vi "Test Running Entry.vi"(8 "error in (no error)":errorcluster, 10 "Work Folder":path, 11 "Test Data Folder":path) -> (0 "error out":errorcluster, 2 "Report":string, 3 "Passed":bool)   [LabVIEW 2024]
doc: "A running entry has End Time 0 in memory and End Time = \"\" in the file. Saves an entry that started an hour ago with no end and checks that Get Running Entry returns it, that the file holds End Time = \"\" and that Read Entry gives End Time 0 back. Then checks the other direction with the README sample: its entry with End Time = \"\" (Nov 2025) is found as running by Find Running Entry.vi when Now is 15 Nov 2025.\n\nInputs: Test Data Folder holds the source copies (Samples, v1); each run works in a new case folder under Work Folder. Passed is TRUE when every check passed and no error occurred; Report lists every check.\n\nGenerated by: Claude"
uses:
  Storage/Project Store-INI/Project Store-INI.lvclass
  Storage/Time Entry Store-INI/Time Entry Store-INI.lvclass
  Utilities/Time Management/Time Management.lvlib
  Storage/Time Entry Store/Time Entry Store.lvclass
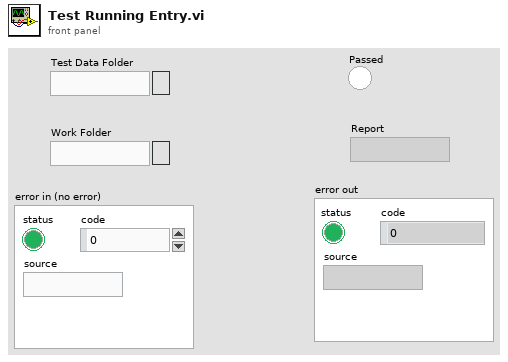
[diagram p1: front panel]
types:
  T1 = cluster{"c6021":string, "c6022":string, "c6023":string, timestamp, "Timestamp":timestamp, "c6024":string}
  T2 = typedef "Time Entry.ctl" = cluster{"ID":string, "Project ID":string, "Task ID":string, "Start Time":timestamp, "End Time":timestamp, "Description":string}
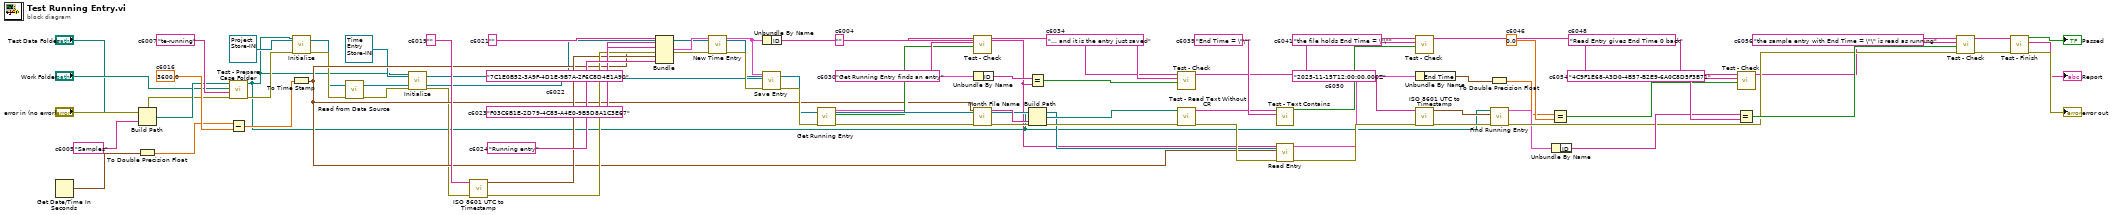
[diagram p0: block diagram]
diagram:
  w72 = "the sample entry with End Time = \"\" is read as running"  # c6056
  w70 = "4C9F1E68-A3D0-4B57-B2E9-6A0C8D5F3B71"  # c6054
  w64 = "2025-11-15T12:00:00.000Z"  # c6050
  w62 = "Read Entry gives End Time 0 back"  # c6048
  w60 = 0.0  # c6046
  w54 = "the file holds End Time = \"\""  # c6041
  w52 = "End Time = \"\""  # c6039
  w45 = "... and it is the entry just saved"  # c6034
  w41 = "Get Running Entry finds an entry"  # c6030
  w29 = "Running entry"  # c6024
  w28 = "F03C6B1E-2D79-4C85-A4E0-9B5D8A1C3E67"  # c6023
  w27 = "7C1E0B52-3A9F-4D1E-9B7A-2F6C8D4E1A90"  # c6022
  w26 = ""  # c6021
  w23 = ""  # c6019
  w20 = 3600.0  # c6016
  w7 = "te-running"  # c6007
  w5 = "Samples"  # c6005
  w4 = ""  # c6004
  n1 = Get Date/Time In Seconds() -> (seconds since 1Jan1904=w18:timestamp)
  n2 = Build Path(base path="Test Data Folder", name or relative path=w5) -> (appended path=w6:path)
  n3 = To Double Precision Float(number=w18) -> (double precision float=w19:dbl)
  n4 = call "Test - Prepare Case Folder.vi"("error in (no error)"="error in (no error)", "Case Name"=w7, "Work Folder"="Work Folder", "Source Folder"=w6) -> ("error out"=w9:errorcluster, "Case Folder"=w8:path)  [unwired: 6 in]
  n5 = Subtract(x=w19, y=w20) -> (x-y=w21:dbl)
  n6 = call-dynamic "Initialize.vi"("Project Store in"=refnum<class "Project Store-INI.lvclass"> refnum ("Project Store-INI"), "error in (no error)"=w9, "Data Folder"=w8) -> ("error out"=w12:errorcluster, "Project Store out"=w11:refnum<class "Project Store-INI.lvclass">)  [unwired: 7 in]
  n7 = To Time Stamp(1:w21) -> (0:w22:timestamp)
  n8 = call-dynamic "Read from Data Source.vi"("Project Store in"=w11, "error in (no error)"=w12) -> ("error out"=w14:errorcluster, "Project Store out"=w13:refnum<class "Project Store-INI.lvclass">)  [unwired: 8 in]
  n9 = call-dynamic "Initialize.vi"("Time Entry Store in"=refnum<class "Time Entry Store-INI.lvclass"> refnum ("Time Entry Store-INI"), "error in (no error)"=w14, "Data Folder"=w8) -> ("error out"=w17:errorcluster, "Time Entry Store out"=w16:refnum<class "Time Entry Store-INI.lvclass">)  [unwired: 7 in]
  n10 = call "ISO 8601 UTC to Timestamp.vi"("error in (no error)"=w17, "ISO 8601 UTC"=w23) -> ("error out"=w25:errorcluster, "Timestamp"=w24:timestamp)  [unwired: 8 in]
  n11 = Bundle("c6021"=w26, "c6022"=w27, "c6023"=w28, w22, "Timestamp"=w24, "c6024"=w29) -> (w30:T1)  [unwired: 1 in]
  n12 = call "New Time Entry.vi"("Time Entry Store in"=w16, "error in (no error)"=w25, "Time Entry"=w30) -> ("error out"=w33:errorcluster, "New Time Entry"=w31:T2, "Time Entry Store out"=w32:refnum<class "Time Entry Store-INI.lvclass">)  [unwired: 6 in]
  n13 = Unbundle By Name(w31) -> ("ID"=w34:string)
  n14 = call-dynamic "Save Entry.vi"("Time Entry Store in"=w32, "error in (no error)"=w33, "Project Store"=w13, "Time Entry"=w31) -> ("error out"=w36:errorcluster, "Time Entry Store out"=w35:refnum<class "Time Entry Store-INI.lvclass">)  [unwired: 6 in]
  n15 = call-dynamic "Get Running Entry.vi"("Time Entry Store in"=w35, "error in (no error)"=w36) -> ("error out"=w40:errorcluster, "found?"=w38:bool, "Time Entry"=w37:T2, "Time Entry Store out"=w39:refnum<class "Time Entry Store-INI.lvclass">)  [unwired: 6 in]
  n16 = call "Test - Check.vi"("Condition"=w38, "Check Name"=w41, "Report in"=w4) -> ("Report out"=w42:string)  [unwired: 7 in, 1 out]
  n17 = Unbundle By Name(w37) -> ("ID"=w43:string)
  n18 = call "Month File Name.vi"("error in (no error)"=w40, "Start Time"=w22) -> ("error out"=w48:errorcluster, "File Name"=w47:string)  [unwired: 8 in]
  n19 = Equal?(x=w43, y=w34) -> (x = y?=w44:bool)
  n20 = Build Path(base path=w8, name or relative path=w47) -> (appended path=w49:path)
  n21 = call "Test - Check.vi"("Condition"=w44, "Check Name"=w45, "Report in"=w42) -> ("Report out"=w46:string)  [unwired: 7 in, 1 out]
  n22 = call "Test - Read Text Without CR.vi"("error in (no error)"=w48, "File"=w49) -> ("error out"=w51:errorcluster, "Text"=w50:string)  [unwired: 8 in]
  n23 = call "Test - Text Contains.vi"("Search Text"=w52, "Text"=w50) -> ("Contains?"=w53:bool)  [unwired: 8 in, 1 out]
  n24 = call-dynamic "Read Entry.vi"("Time Entry Store in"=w39, "error in (no error)"=w51, "Start Time"=w22, "ID"=w34) -> ("error out"=w57:errorcluster, "Time Entry"=w56:T2)  [unwired: 4 in, 2 out]
  n25 = call "Test - Check.vi"("Condition"=w53, "Check Name"=w54, "Report in"=w46) -> ("Report out"=w55:string)  [unwired: 7 in, 1 out]
  n26 = Unbundle By Name(w56) -> ("End Time"=w58:timestamp)
  n27 = call "ISO 8601 UTC to Timestamp.vi"("error in (no error)"=w57, "ISO 8601 UTC"=w64) -> ("error out"=w66:errorcluster, "Timestamp"=w65:timestamp)  [unwired: 8 in]
  n28 = To Double Precision Float(number=w58) -> (double precision float=w59:dbl)
  n29 = call "Find Running Entry.vi"("error in (no error)"=w66, "Now"=w65, "Data Folder"=w8) -> ("error out"=w68:errorcluster, "Time Entry"=w67:T2)  [unwired: 6 in, 1 out]
  n30 = Equal?(x=w59, y=w60) -> (x = y?=w61:bool)
  n31 = Unbundle By Name(w67) -> ("ID"=w69:string)
  n32 = call "Test - Check.vi"("Condition"=w61, "Check Name"=w62, "Report in"=w55) -> ("Report out"=w63:string)  [unwired: 7 in, 1 out]
  n33 = Equal?(x=w69, y=w70) -> (x = y?=w71:bool)
  n34 = call "Test - Check.vi"("Condition"=w71, "Check Name"=w72, "Report in"=w63) -> ("Report out"=w73:string)  [unwired: 7 in, 1 out]
  n35 = call "Test - Finish.vi"("error in (no error)"=w68, "Report"=w73) -> ("error out"=→"error out":errorcluster, "Report out"=→"Report":string, "Passed"=→"Passed":bool)  [unwired: 7 in]
